vi "Loop Async.vi"(10 "ExecAnchor":refnum<class "ExecAnchor.lvclass">, 11 "Basic WebSocket Manager in":refnum<class "Basic WebSocket Manager.lvclass">) -> ()   [LabVIEW 2020, in "HTTP Server.lvlib" / "Basic WebSocket Manager.lvclass"]
uses:
  Basic WebSocket Manager.lvclass
  lv-exec-anchor/ExecAnchor/ExecAnchor.lvclass
  WebSocket Client/WebSocket Client.lvclass
  Basic WebSocket Manager.lvclass/Basic WebSocket Manager.ctl
  WebSocket Client/WebSocket Client.lvclass/WebSocket Client.ctl
  lv-http-util/HTTP Utils/Request/Request.lvclass/Request.ctl
  lv-uri/URI/URI/URI.lvclass/URI.ctl
  lv-http-util/HTTP Utils/Request/Get Client URI.vi
  lv-uri/URI/URI/URI String.vi
  lv-uri/URI/Build URI String.vi
  lv-uri/URI/Build Query String.vi
  lv-promises/Promises/Promise/Promise.lvclass
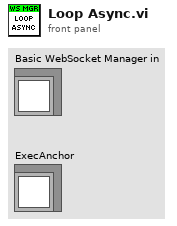
[diagram p1: front panel]
types:
  T1 = map{string, refnum<class "WebSocket Client.lvclass">}
  T2 = cluster{"Event Reg":refnum<event-registration>, "Event Reg":refnum<event-registration>}
  T3 = typedef "HTTP Server.lvlib/WebSocket Format.ctl" = enum16{"Text", "Binary"}
  T4 = cluster{"Client URI String":string, "Format":T3, "Payload":string}
  T5 = typedef "HTTP Server.lvlib/Basic WebSocket Manager.lvclass/Ref Data.ctl" = cluster{"Clients":map{string, refnum<class "WebSocket Client.lvclass">}}
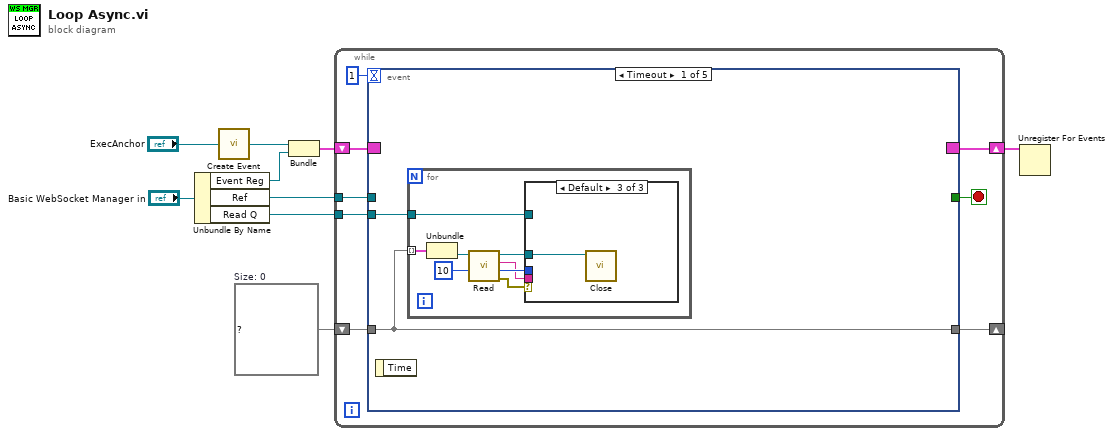
[diagram p0: block diagram]
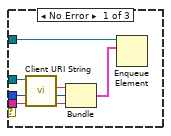
[diagram p2: hidden frame]
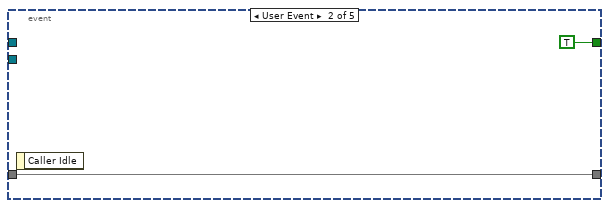
[diagram p4: hidden frame]
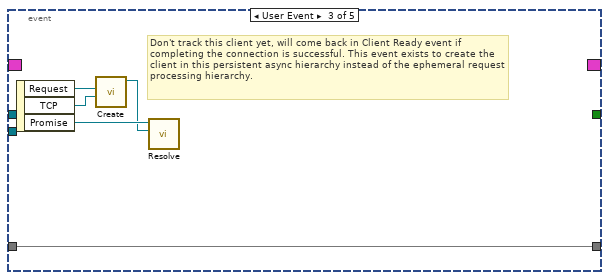
[diagram p5: hidden frame]
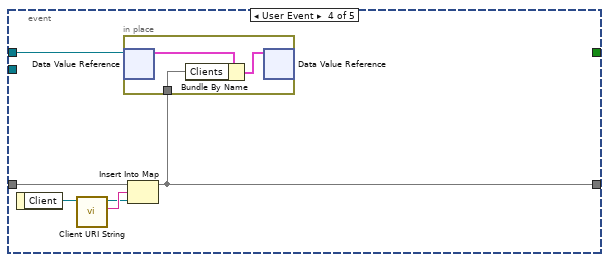
[diagram p6: hidden frame]
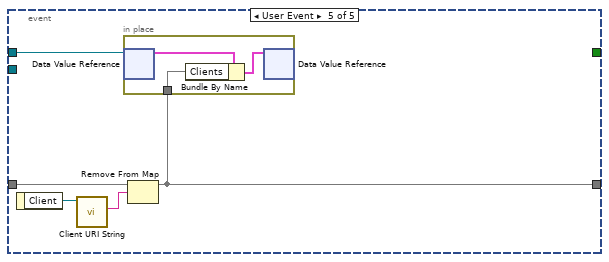
[diagram p7: hidden frame]
diagram:
  w3 = T1 {}  # Size: 0
  n1 = Unbundle By Name("Basic WebSocket Manager in") -> ("Event Reg"=w6:refnum<event-registration>, "Ref"=w2:refnum<data-value>, "Read Q"=w1:refnum<queue>)
  n2 = call "Create Event.vi"("ExecAnchor in"="ExecAnchor") -> ("Event Reg"=w7:refnum<event-registration>)  [unwired: 3 in, 1 out]
  n3 = Bundle("Event Reg"=w7, "Event Reg"=w6) -> (w5:T2)  [unwired: 1 in]
  n4 = while {
    shift-right: [w16] -> w4
    shift-left: w5 -> [w17]
    shift-right: [w13] -> _
    shift-left: w3 -> [w14]
    tunnel: w2 -> [w12]
    tunnel: w1 -> [w10]
    stop <- w15 stop-if-true
    n5 = event shown="[0] Timeout" {
      selector: w17 -> [_ _ _ _ _]
      dyn-events: [_ _ _ _ _] -> w16
      timeout: 1 -> [_ _ _ _ _]
      tunnel: [_ TRUE _ _ _] -> w15
      tunnel: w14 -> [w19 w35 w37 w47 w54]
      tunnel: [w19 w35 w37 w42 w51] -> w13
      tunnel: w12 -> [_ _ _ w43 w52]
      tunnel: w10 -> [w18 _ _ _ _]
      event Timeout {
        n6 = event-data() -> ()  [unwired: 1 in, 1 out]
        n7 = for {
          tunnel: w19 -> [w27] mode=indexing
          tunnel: w18 -> [w23]
          n8 = Unbundle(w27) -> ("HTTP Server:WebSocket Client.lvclass"=w26:refnum<class "WebSocket Client.lvclass">)  [unwired: 1 out]
          n9 = call "Read.vi"("Timeout ms (1000)"=10, "WebSocket Client in"=w26) -> ("error out"=w24:errorcluster, "Format"=w22:T3, "Payload"=w21:string, "WebSocket Client out"=w20:refnum<class "WebSocket Client.lvclass">)  [unwired: 6 in]
          n10 = case shown="Default" w24 {
            tunnel: w23 -> [w33 _ _]
            tunnel: w22 -> [w32 _ _]
            tunnel: w21 -> [w31 _ _]
            tunnel: w20 -> [w29 _ w34]
            frame No Error {
              n11 = call "Client URI String.vi"("WebSocket Client in"=w29) -> ("Client URI String"=w28:string)  [unwired: 9 in, 1 out]
              n12 = Bundle("Client URI String"=w28, "Format"=w32, "Payload"=w31) -> (w30:T4)  [unwired: 1 in]
              n13 = Enqueue Element(queue=w33, element=w30) -> ()  [unwired: 2 in, 3 out]
            }
            frame Error {
            }
            frame Default {
              n14 = call "Close.vi"("WebSocket Client in"=w34) -> ()  [unwired: 9 in, 2 out]
            }
          }
        }
      }
      event User Event {
        n15 = event-data() -> ()  [unwired: 1 in, 1 out]
      }
      event User Event {
        # "Don't track this client yet, will come back in Client Ready event if completing the connection is successful. This event exists to create the client in this persistent async hierarchy instead of the ephemeral request processing hierarchy."
        n16 = event-data() -> ("Request"=w41:refnum<class "Request.lvclass">, "TCP"=w40:refnum<k5>, "Promise"=w39:refnum<class "Promise.lvclass">)  [unwired: 1 in]
        n17 = call "Create.vi"("TCP"=w40, "Request"=w41) -> ("WebSocket Client out"=w38:refnum<class "WebSocket Client.lvclass">)  [unwired: 8 in, 1 out]
        n18 = call "Resolve.vi"("Result (None)"=w38, "Promise in"=w39) -> ()  [unwired: 8 in, 2 out]
      }
      event User Event {
        n19 = event-data() -> ("Client"=w46:refnum<class "WebSocket Client.lvclass">)  [unwired: 1 in]
        n20 = call "Client URI String.vi"("WebSocket Client in"=w46) -> ("Client URI String"=w45:string, "WebSocket Client out"=w44:refnum<class "WebSocket Client.lvclass">)  [unwired: 9 in]
        n21 = Insert Into Map(map in=w47, key=w45, value=w44) -> (map out=w42:T1)  [unwired: 2 out]
        n22 = in-place {
          in-place-border: w42 -> [w49]
          n23 = in-place-dvr #1(w43) -> (w50:T5)  [unwired: 1 out]
          n24 = Bundle By Name(cluster=w50, "Clients"=w49) -> (w48:T5)
          n25 = in-place-dvr #1(w48) -> ()  [unwired: 2 out]
        }
      }
      event User Event {
        n26 = event-data() -> ("Client"=w55:refnum<class "WebSocket Client.lvclass">)  [unwired: 1 in]
        n27 = call "Client URI String.vi"("WebSocket Client in"=w55) -> ("Client URI String"=w53:string)  [unwired: 9 in, 1 out]
        n28 = Remove From Map(10:w53, 11:w54) -> (3:w51:T1)  [unwired: 2 out]
        n29 = in-place {
          in-place-border: w51 -> [w57]
          n30 = in-place-dvr #2(w52) -> (w58:T5)  [unwired: 1 out]
          n31 = Bundle By Name(cluster=w58, "Clients"=w57) -> (w56:T5)
          n32 = in-place-dvr #2(w56) -> ()  [unwired: 2 out]
        }
      }
    }
  }
  n33 = Unregister For Events(event registration refnum=w4) -> ()  [unwired: 1 in, 1 out]
